vi "entry_stopped.vi"() -> ()   [LabVIEW 2012]
panel:
  out "Telemetry stop enqueue timed out 2":bool
  out "Telemetry stop enqueue timed out 1":bool
  out "Telemetry stop enqueue error 2":errorcluster caption="sortie d'erreur"
  out "Telemetry stop enqueue error 1":errorcluster caption="sortie d'erreur"
  out "Camera stop queue cleanup error":errorcluster caption="sortie d'erreur"
  out "Camera data queue cleanup error":errorcluster caption="sortie d'erreur"
  out "Telemetry startup error":errorcluster caption="sortie d'erreur"
  out "Queue cleanup error 2":errorcluster caption="sortie d'erreur"
  out "Queue cleanup error":errorcluster caption="sortie d'erreur"
  in  "packet":variant
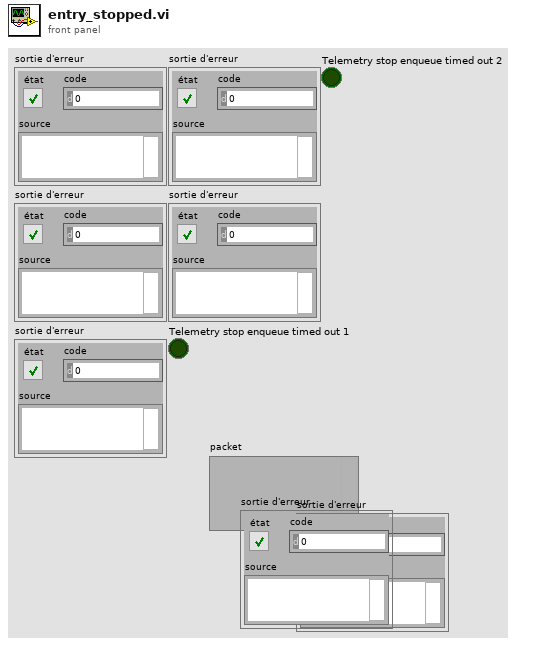
[diagram p1: front panel]
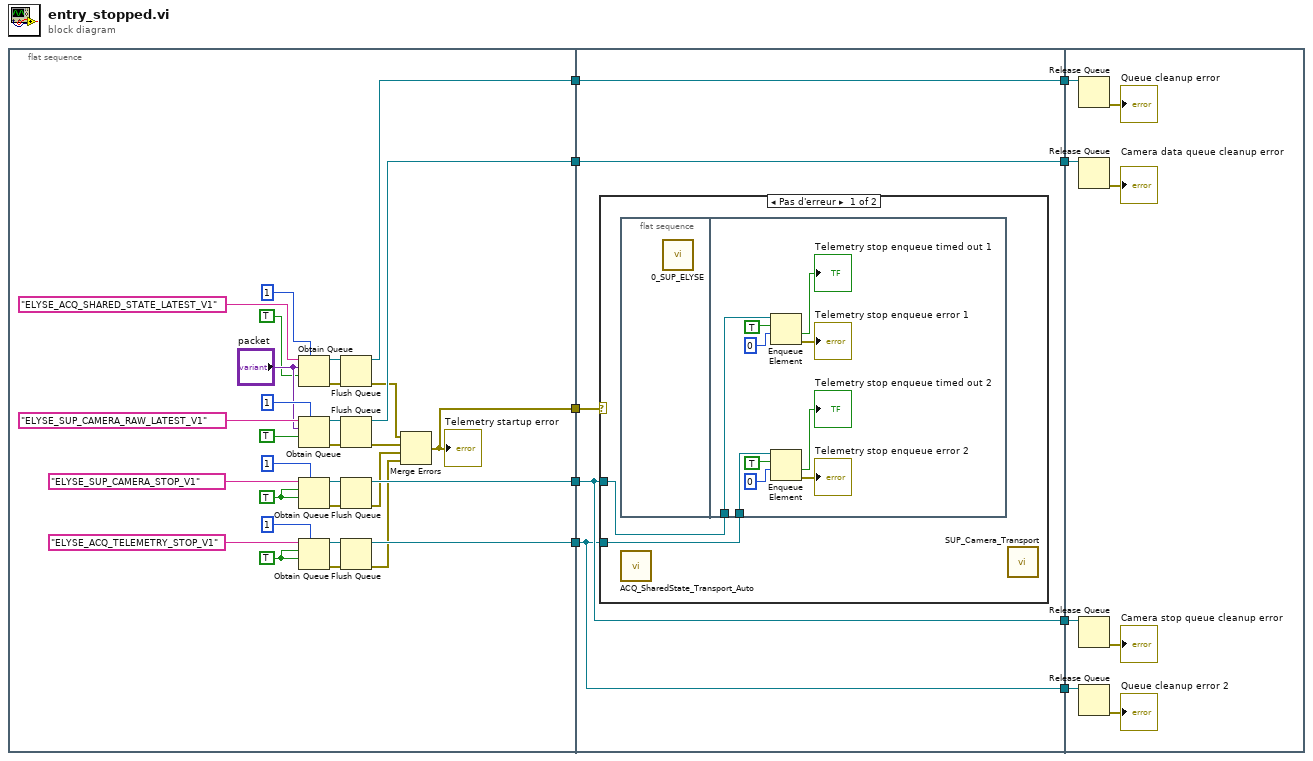
[diagram p0: block diagram]
diagram:
  n1 = flat-sequence {
    tunnel: [w19] -> w4
    tunnel: [w21] -> w2
    tunnel: [w20] -> w8
    tunnel: [w31] -> w6
    tunnel: [w14] -> w1
    tunnel: [w42] -> w5
    tunnel: w4 -> [w42]
    tunnel: [w41] -> w3
    tunnel: w2 -> [w41]
    tunnel: [w44] -> w9
    tunnel: w8 -> [w44]
    tunnel: [w43] -> w7
    tunnel: w6 -> [w43]
    tunnel: w1 -> [w40]
    tunnel: w5 -> [w60]
    tunnel: w3 -> [w59]
    tunnel: w9 -> [w64]
    tunnel: w7 -> [w63]
    frame #0 {
      w34 = TRUE ("créer si introuvable ? (V)")
      w24 = TRUE ("créer si introuvable ? (V)")
      n2 = Obtain Queue(max queue size (-1, unlimited)=1 ("taille max de la file d'attente (-1, non limitée)"), name (unnamed)="ELYSE_ACQ_SHARED_STATE_LATEST_V1" ("nom (aucun)"), element data type="packet", create if not found? (T)=TRUE ("créer si introuvable ? (V)")) -> (queue out=w22:refnum<queue>, error out=w11:errorcluster)  [unwired: 1 in, 1 out]
      n3 = Obtain Queue(max queue size (-1, unlimited)=1 ("taille max de la file d'attente (-1, non limitée)"), name (unnamed)="ELYSE_SUP_CAMERA_RAW_LATEST_V1" ("nom (aucun)"), element data type="packet", create if not found? (T)=TRUE ("créer si introuvable ? (V)")) -> (queue out=w32:refnum<queue>, error out=w10:errorcluster)  [unwired: 1 in, 1 out]
      n4 = Obtain Queue(max queue size (-1, unlimited)=1 ("taille max de la file d'attente (-1, non limitée)"), name (unnamed)="ELYSE_SUP_CAMERA_STOP_V1" ("nom (aucun)"), element data type=w34, create if not found? (T)=w34) -> (queue out=w33:refnum<queue>, error out=w13:errorcluster)  [unwired: 1 in, 1 out]
      n5 = Obtain Queue(max queue size (-1, unlimited)=1 ("taille max de la file d'attente (-1, non limitée)"), name (unnamed)="ELYSE_ACQ_TELEMETRY_STOP_V1" ("nom (aucun)"), element data type=w24, create if not found? (T)=w24) -> (queue out=w23:refnum<queue>, error out=w12:errorcluster)  [unwired: 1 in, 1 out]
      n6 = Flush Queue(queue=w22, error in (no error)=w11) -> (queue out=w19:refnum<queue>, error out=w18:errorcluster)  [unwired: 1 out]
      n7 = Flush Queue(queue=w32, error in (no error)=w10) -> (queue out=w20:refnum<queue>, error out=w17:errorcluster)  [unwired: 1 out]
      n8 = Flush Queue(queue=w33, error in (no error)=w13) -> (queue out=w31:refnum<queue>, error out=w16:errorcluster)  [unwired: 1 out]
      n9 = Flush Queue(queue=w23, error in (no error)=w12) -> (queue out=w21:refnum<queue>, error out=w15:errorcluster)  [unwired: 1 out]
      n10 = Merge Errors(w18, w17, w16, w15) -> (w14:errorcluster)
      "Telemetry startup error" <- w14
    }
    frame #1 {
      n11 = case shown="Pas d'erreur" w40 {
        tunnel: w43 -> [w46 _]
        tunnel: w41 -> [w45 _]
        frame No Error {
          n12 = flat-sequence {
            tunnel: w45 -> [w53]
            tunnel: w46 -> [w56]
            frame #0 {
              n13 = call "0_SUP_ELYSE.vi"() -> ()  [unwired: 1 in]
            }
            frame #1 {
              n14 = Enqueue Element(queue=w56, element=TRUE ("élément"), timeout in ms (-1)=0 ("timeout en ms (-1)")) -> (timed out?=→"Telemetry stop enqueue timed out 1":bool, error out=→"Telemetry stop enqueue error 1":errorcluster)  [unwired: 1 in, 1 out]
              n15 = Enqueue Element(queue=w53, element=TRUE ("élément"), timeout in ms (-1)=0 ("timeout en ms (-1)")) -> (timed out?=→"Telemetry stop enqueue timed out 2":bool, error out=→"Telemetry stop enqueue error 2":errorcluster)  [unwired: 1 in, 1 out]
            }
          }
          n16 = call "ACQ_SharedState_Transport_Auto.vi"() -> ()  [unwired: 12 in]
          n17 = call "SUP_Camera_Transport.vi"() -> ()  [unwired: 12 in]
        }
        frame Error {
        }
      }
    }
    frame #2 {
      n18 = Release Queue(queue=w60) -> (error out=→"Queue cleanup error":errorcluster)  [unwired: 2 in, 2 out]
      n19 = Release Queue(queue=w64) -> (error out=→"Camera data queue cleanup error":errorcluster)  [unwired: 2 in, 2 out]
      n20 = Release Queue(queue=w63) -> (error out=→"Camera stop queue cleanup error":errorcluster)  [unwired: 2 in, 2 out]
      n21 = Release Queue(queue=w59) -> (error out=→"Queue cleanup error 2":errorcluster)  [unwired: 2 in, 2 out]
    }
  }
